vi "CreateMethodNames.vi"(0 "_Method":i32[](array[numeric]), 1 "FileNamingOption":T1, 2 "_Property":string[](array[string]), 3 "Item Names":string[](array[string]), 4 "Use Read/Write":bool) -> (5 "MethodNames":string[](array[string]), 6 "Attribute/PropertyNames":string[](array[string]))   [LabVIEW 2020, in "ClassWriterNative.lvclass"]
uses:
  <resource>/Framework/Providers/Open_GDS/ClassProviders/Provider_LvNativeClass/ClassWriterNative_class/ClassWriterNative.lvclass
  <resource>/Framework/Providers/Open_GDS/ClassProviders/Provider_BaseClassInterface/BaseProvider_SubVIs/BaseProvider_FileNamingOption.ctl
  <resource>/Framework/Providers/Open_GDS/ClassProviders/Provider_LvNativeClass/ClassWriterNative_class/ClassWriterNative.lvclass/ClassWriterNative.ctl
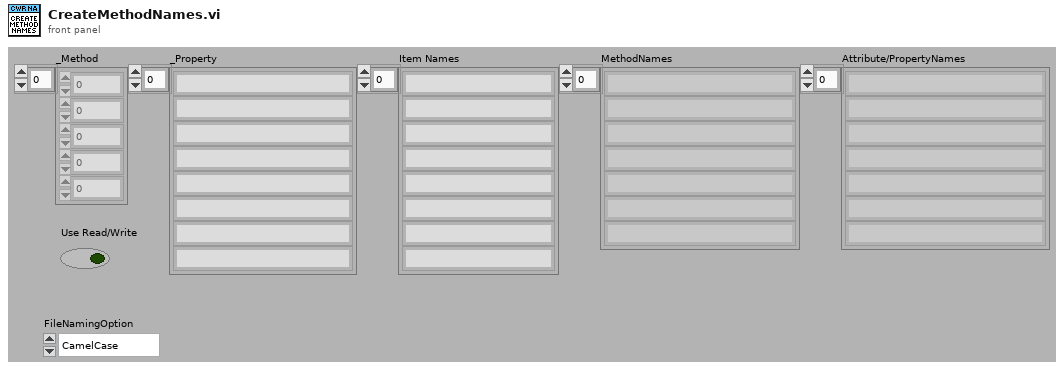
[diagram p1: front panel]
types:
  T1 = typedef "BaseProvider_FileNamingOption.ctl" = enum16{"CamelCase", "Space", "Underscore"}
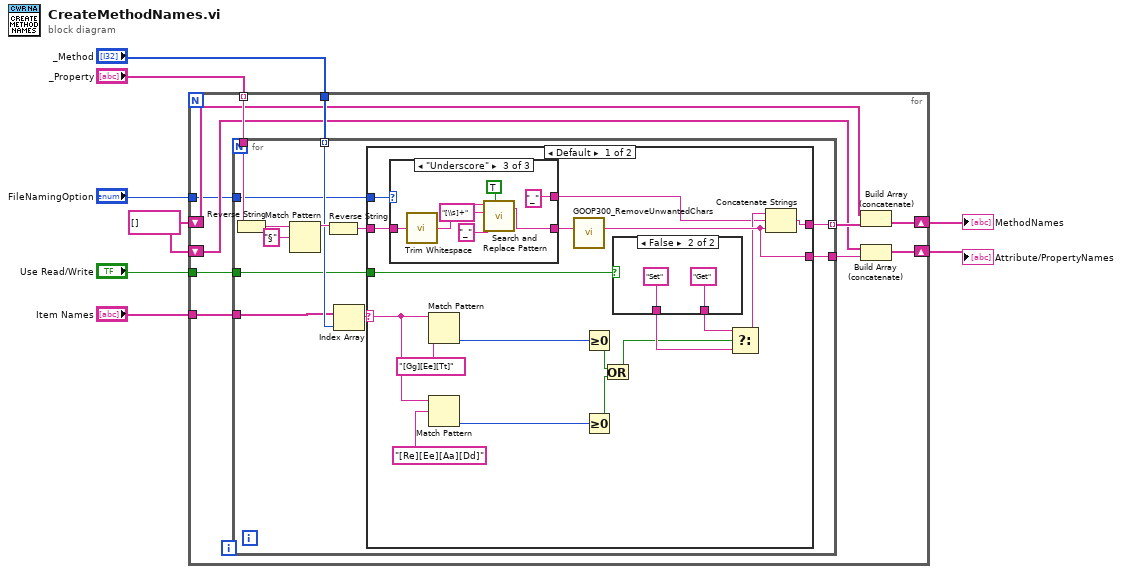
[diagram p0: block diagram]
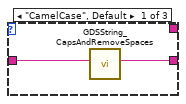
[diagram p2: hidden frame]
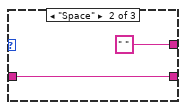
[diagram p3: hidden frame]
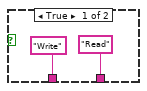
[diagram p4: hidden frame]
diagram:
  w3 = string[] []
  n1 = for {
    tunnel: "_Property" -> [w19] mode=indexing
    tunnel: "_Method" -> [w18]
    shift-right: [w16] -> w8
    shift-left: w3 -> [w15]
    tunnel: "Item Names" -> [w14]
    tunnel: "Use Read/Write" -> [w13]
    shift-right: [w12] -> w2
    shift-left: w3 -> [w10]
    tunnel: "FileNamingOption" -> [w9]
    n2 = for {
      tunnel: w19 -> [w31]
      tunnel: w18 -> [w25] mode=indexing
      tunnel: [w24] -> w17 mode=indexing
      tunnel: w14 -> [w23]
      tunnel: w13 -> [w22]
      tunnel: [w21] -> w11
      tunnel: w9 -> [w20]
      n3 = Reverse String(1:w31) -> (0:w30:string)
      n4 = Match Pattern(string=w30, regular expression="§") -> (before substring=w28:string)  [unwired: 1 in, 3 out]
      n5 = Reverse String(1:w28) -> (0:w26:string)
      n6 = Index Array(array=w23, index=w25) -> (element=w27:string)
      n7 = case shown="Default" w27 {
        selector: w27 -> [w41 _]
        tunnel: w26 -> [w45 _]
        tunnel: [w43 _] -> w24
        tunnel: w22 -> [w35 _]
        tunnel: [w36 _] -> w21
        tunnel: w20 -> [w34 _]
        frame Default {
          n8 = case shown="\"Underscore\"" w34 {
            tunnel: w45 -> [w51 w53 w60]
            tunnel: [w50 w53 w57] -> w44
            tunnel: [_ " " "_"] -> w32
            frame "CamelCase", Default {
              n9 = call <resource>:"GDSString_CapsAndRemoveSpaces.vi"("String"=w51) -> ("concatenated string"=w50:string)  [unwired: 10 in]
            }
            frame "Space" {
            }
            frame "Underscore" {
              n10 = call <vilib>:"Trim Whitespace.vi"("string"=w60) -> ("trimmed string"=w56:string)  [unwired: 1 in]
              n11 = call <vilib>:"Search and Replace Pattern.vi"("string"=w56, "regular expression (\"\")"="[\\s]+" ("regular expression (\"\")"), "replace string (\"\")"="_" ("replace string (\"\")"), "replace all? (F)"=TRUE) -> ("result string"=w57:string)  [unwired: 1 in, 1 out]
            }
          }
          n12 = Match Pattern(string=w41, regular expression="[Gg][Ee][Tt]") -> (offset past match=w48:i32)  [unwired: 1 in, 3 out]
          n13 = Match Pattern(string=w41, regular expression="[Re][Ee][Aa][Dd]") -> (offset past match=w40:i32)  [unwired: 1 in, 3 out]
          n14 = call <resource>:"GOOP300_RemoveUnwantedChars.vi"("StringIn"=w44) -> ("StringOut"=w36:string)  [unwired: 10 in]
          n15 = Greater Or Equal To 0?(x=w48) -> (x >= 0?=w38:bool)
          n16 = Greater Or Equal To 0?(x=w40) -> (x >= 0?=w39:bool)
          n17 = Or(x=w38, y=w39) -> (x .or. y?=w37:bool)
          n18 = case shown="False" w35 {
            tunnel: ["Read" ("regular expression") "Get" ("regular expression")] -> w47
            tunnel: ["Write" ("regular expression") "Set" ("regular expression")] -> w46
            frame True {
            }
            frame False {
            }
          }
          n19 = Select(t=w47, s=w37, f=w46) -> (s? t:f=w33:string)
          n20 = Concatenate Strings(w33, w32, w36) -> (w43:string)
        }
        frame "" {
        }
      }
    }
    n21 = Build Array (concatenate)(w15, w17) -> (w16:string[])
    n22 = Build Array (concatenate)(w10, w11) -> (w12:string[])
  }
  "MethodNames" <- w8
  "Attribute/PropertyNames" <- w2
